vi "Version.vi"(8 "error in (no error)":errorcluster) -> (0 "error out":errorcluster, 1 "version (str)":string, 2 "minor":i32, 3 "mayor":i32)   [LabVIEW 2020, in "wiringPi.lvlib"]
doc: "<b>_______________________________________________________________</b>\n** Author: Juan José Villacorta\n** LabVIEW wrapper for C library <b> wiringPi </b>,\n** https://github.com/WiringPi/WiringPi\n<b>_______________________________________________________________</b>\n\n\n/*\n * wiringPiVersion:\n * Return our current version number\n *********************************************************************************\n */"
uses:
  wiringPi.lvlib
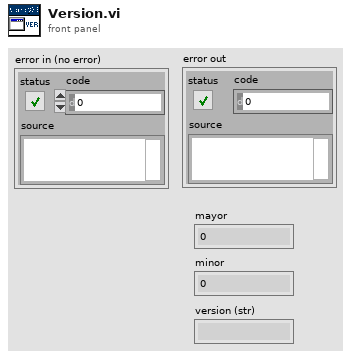
[diagram p1: front panel]
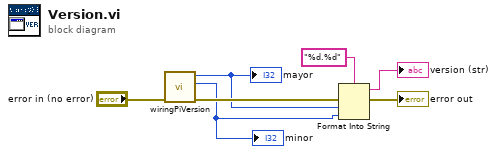
[diagram p0: block diagram]
diagram:
  n1 = call "wiringPiVersion.vi"("error in (no error)"="error in (no error)") -> ("error out"=w3:errorcluster, "minor"=w1:i32, "mayor"=w2:i32)  [unwired: 8 in]
  "mayor" <- w2
  "minor" <- w1
  n2 = Format Into String(format string="%d.%d", error in=w3, w2, w1) -> (resulting string=→"version (str)":string, error out=→"error out":errorcluster)  [unwired: 1 in]
